vi "GetText.vi"(8 "error in":errorcluster, 11 "TEC editor node in":refnum<class "TEC editor node.lvclass">) -> (0 "error out":errorcluster, 1 "additional text":string, 2 "text":string, 3 "TEC editor node out":refnum<class "TEC editor node.lvclass">, 4 "glyph":string)   [LabVIEW 2013, in "TEC editor node.lvclass"]
uses:
  TEC editor node.lvclass
  <vilib>/NI/DCAF/Tag Editor Core/Configuration Editor/Classes/Module editor node/Read display name.vi
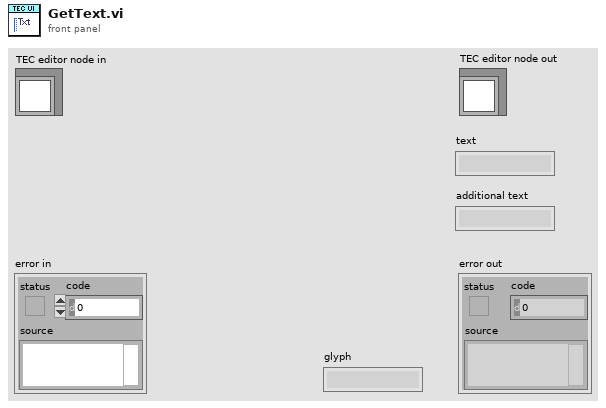
[diagram p1: front panel]
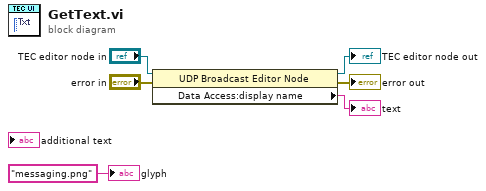
[diagram p0: block diagram]
diagram:
  n1 = property class="UDP Broadcast Editor Node"(reference="TEC editor node in", error in="error in") -> (reference out=→"TEC editor node out":refnum<class "TEC editor node.lvclass">, error out=→"error out":errorcluster, "Data Access:display name"=→"text":string)
  "glyph" <- "messaging.png" ("glyph")
